vi "Get Server Address.vi"(11 "gRPC server in":refnum<class "Servicer.lvclass">) -> (2 "Server Address":string, 3 "gRPC server out":refnum<class "Servicer.lvclass">)   [LabVIEW 2019, in "gRPC-servicer.lvlib" / "Servicer.lvclass"]
uses:
  Servicer.lvclass
  Servicer.lvclass/Servicer.ctl
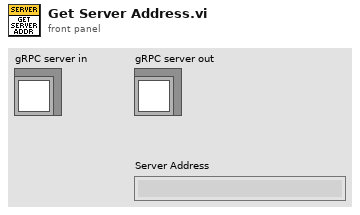
[diagram p1: front panel]
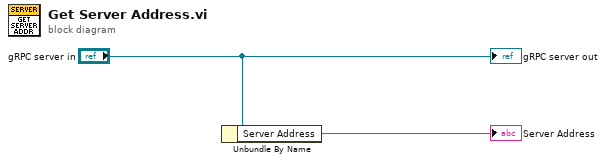
[diagram p0: block diagram]
diagram:
  n1 = Unbundle By Name("gRPC server in") -> ("Server Address"=→"Server Address":string)
  "gRPC server out" <- "gRPC server in"
